vi "KE3706_read_channels_(openvisafirst).vi"(0 "VISA-Ressourcenname":refnum<visa-resource-name>, 7 "Fehler (Eingang, kein Fehler)":errorcluster) -> (12 "Fehler (Ausgang)":errorcluster, 14 "Fehler (Ausgang) 3":errorcluster caption="Fehler (Ausgang)", 18 "Fehler (Ausgang) 6":errorcluster caption="Fehler (Ausgang)", 19 "Display Readings 9":string, 20 "Display Readings":string, 21 "Display Readings 2":string, 22 "Display Readings 3":string, 23 "Display Readings 4":string, 24 "Display Readings 5":string, 25 "Display Readings 6":string, 26 "Display Readings 7":string, 27 "Display Readings 8":string)   [LabVIEW 2020]
panel:
  out "Fehler (Ausgang) 2":errorcluster caption="Fehler (Ausgang)"
  out "Fehler (Ausgang) 9":errorcluster caption="Fehler (Ausgang)"
  out "Fehler (Ausgang) 8":errorcluster caption="Fehler (Ausgang)"
  out "Fehler (Ausgang) 7":errorcluster caption="Fehler (Ausgang)"
  out "Fehler (Ausgang) 5":errorcluster caption="Fehler (Ausgang)"
  out "Fehler (Ausgang) 4":errorcluster caption="Fehler (Ausgang)"
  # "der will eh nie einen Fehler hier ausgeben\nsiehe display da macht er es (manchmal, wenn er will)"
  # "man muss manuel triggern\noder irgendwie mit code\ndas teil ist lustig"
  # "die channel können beide auch ine einem wert ausgegeben werden (mittelwert, wahrscheinlich ka?)\nauf jedenfall muss man darauf achten dass die channel seperat bleiben (?)!\nsollte man das ding überhaupt nutzen\n\nder einzige befehl der keinen error wirft ist gerade drin und selbst mit libs und allem möglicen funktionieren auch keine sample codes aus dem manual\ndas problem mit dem display.gettext() ist dass es sobald das display gelesen wird der automatische trigger ausgeschaltet wird."
  # "^nvm das was jetzt da steht funktioniert auch und funktioniert digital\n\nmuss nur gut voreingestellt werden (jana weiß wie)\n\nEUREKA ES GEHT\n\nGerät function auf mytemp in beiden channels (voreinstellung)"
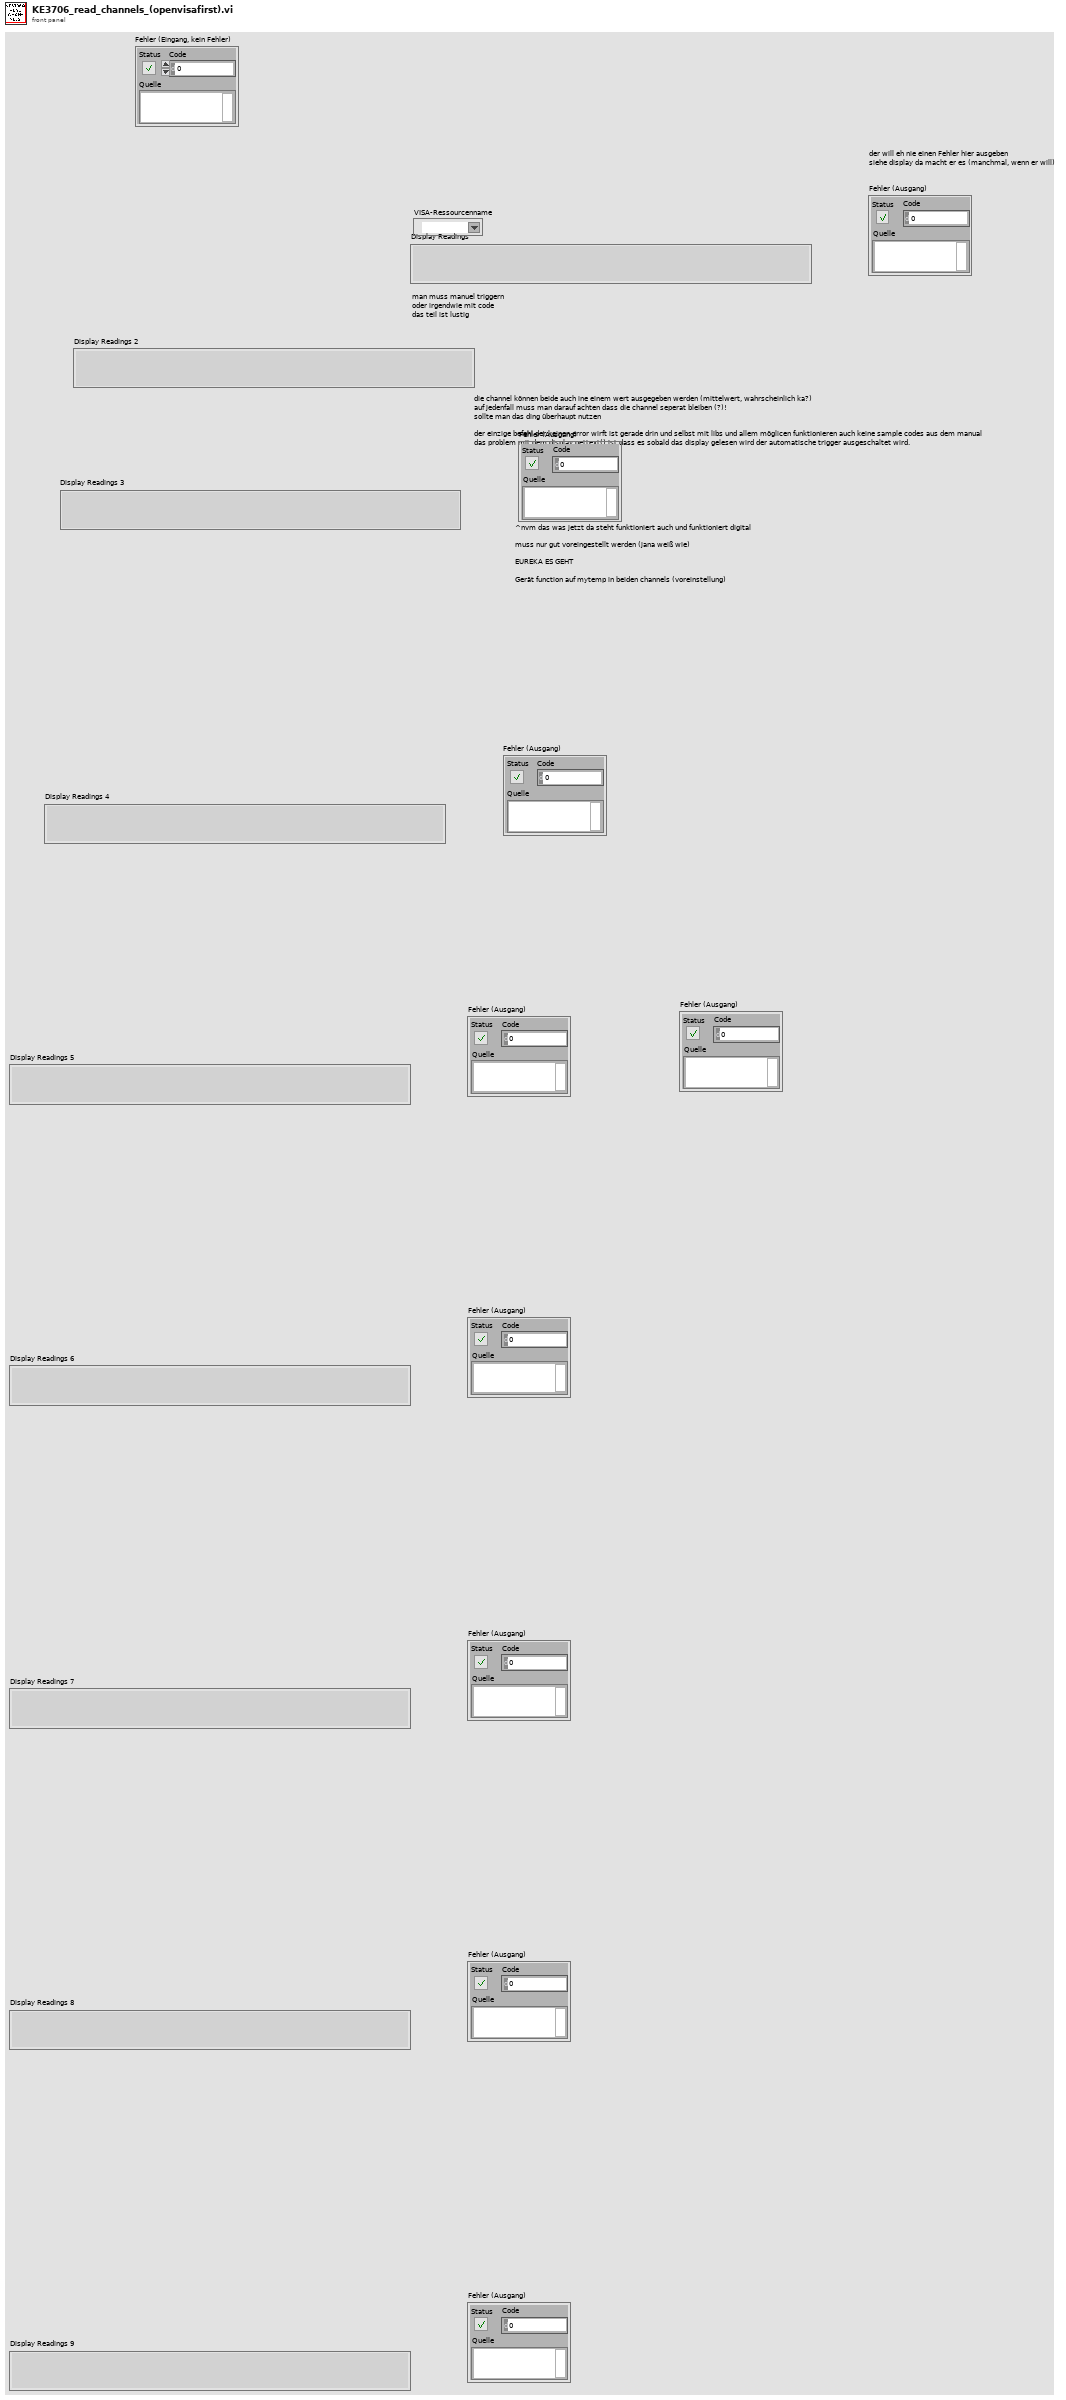
[diagram p1: front panel]
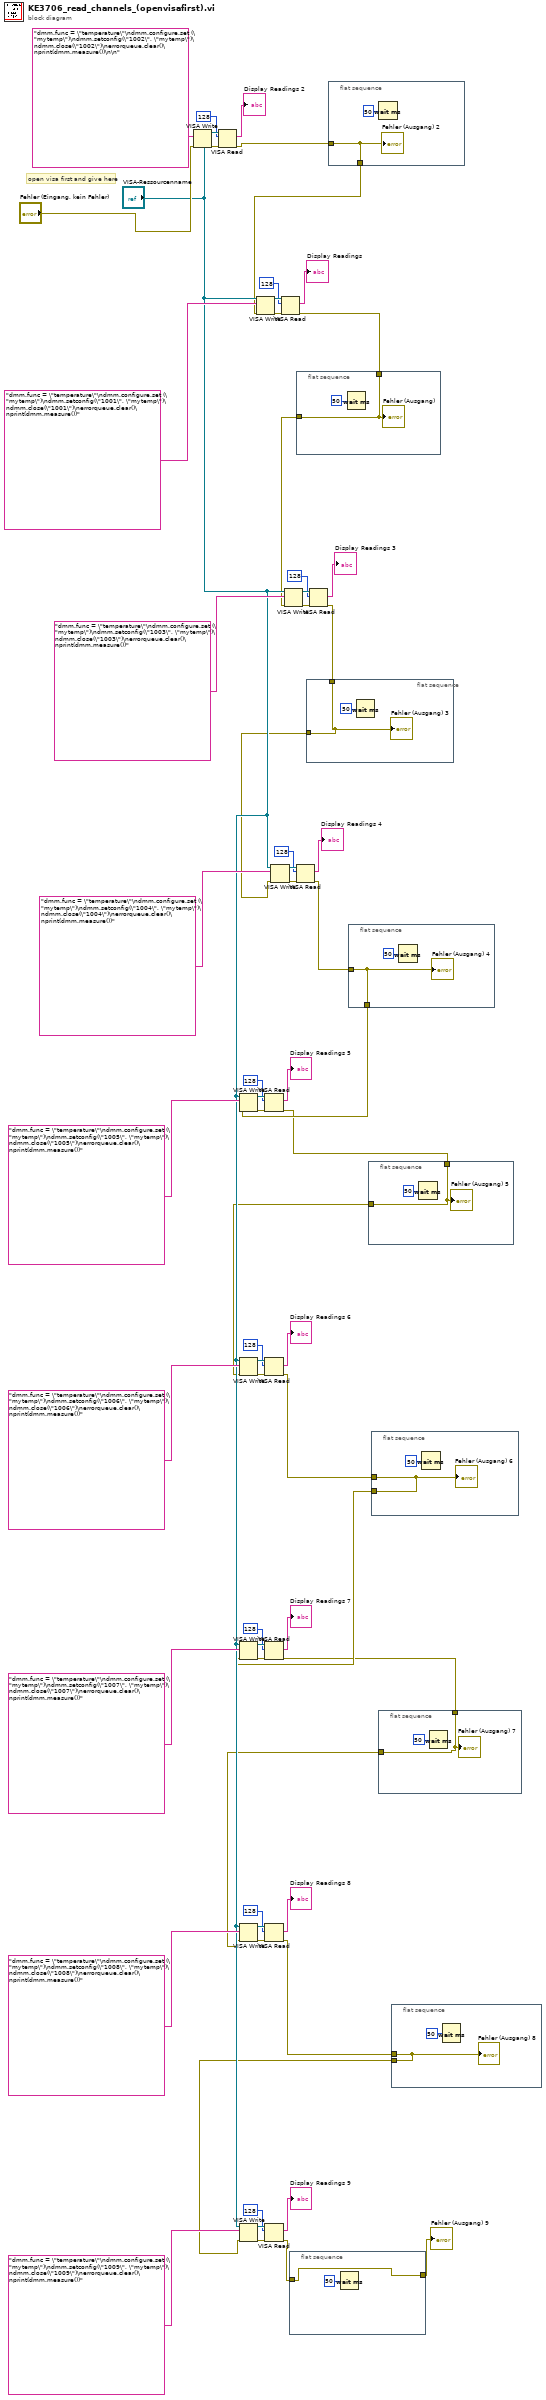
[diagram p0: block diagram]
diagram:
  # "open visa first and give here"
  n1 = VISA Write(VISA resource name="VISA-Ressourcenname", write buffer="dmm.func = \"temperature\"\ndmm.configure.set (\"mytemp\")\ndmm.setconfig(\"1002\", \"mytemp\")\ndmm.close(\"1002\")\nerrorqueue.clear()\nprint(dmm.measure())\n\n" ("Schreibpuffer"), error in (no error)="Fehler (Eingang, kein Fehler)") -> (VISA resource name out=w60:refnum<visa-resource-name>, error out=w59:errorcluster)  [unwired: 1 out]
  n2 = VISA Read(VISA resource name=w60, byte count=u32 128 ("Byte-Anzahl"), error in (no error)=w59) -> (read buffer=→"Display Readings 2":string, error out=w18:errorcluster)  [unwired: 2 out]
  n3 = VISA Write(VISA resource name="VISA-Ressourcenname", write buffer="dmm.func = \"temperature\"\ndmm.configure.set (\"mytemp\")\ndmm.setconfig(\"1005\", \"mytemp\")\ndmm.close(\"1005\")\nerrorqueue.clear()\nprint(dmm.measure())" ("Schreibpuffer"), error in (no error)=w11) -> (VISA resource name out=w44:refnum<visa-resource-name>, error out=w43:errorcluster)  [unwired: 1 out]
  n4 = VISA Write(VISA resource name="VISA-Ressourcenname", write buffer="dmm.func = \"temperature\"\ndmm.configure.set (\"mytemp\")\ndmm.setconfig(\"1006\", \"mytemp\")\ndmm.close(\"1006\")\nerrorqueue.clear()\nprint(dmm.measure())" ("Schreibpuffer"), error in (no error)=w9) -> (VISA resource name out=w39:refnum<visa-resource-name>, error out=w38:errorcluster)  [unwired: 1 out]
  n5 = VISA Write(VISA resource name="VISA-Ressourcenname", write buffer="dmm.func = \"temperature\"\ndmm.configure.set (\"mytemp\")\ndmm.setconfig(\"1007\", \"mytemp\")\ndmm.close(\"1007\")\nerrorqueue.clear()\nprint(dmm.measure())" ("Schreibpuffer"), error in (no error)=w7) -> (VISA resource name out=w34:refnum<visa-resource-name>, error out=w33:errorcluster)  [unwired: 1 out]
  n6 = VISA Write(VISA resource name="VISA-Ressourcenname", write buffer="dmm.func = \"temperature\"\ndmm.configure.set (\"mytemp\")\ndmm.setconfig(\"1008\", \"mytemp\")\ndmm.close(\"1008\")\nerrorqueue.clear()\nprint(dmm.measure())" ("Schreibpuffer"), error in (no error)=w5) -> (VISA resource name out=w29:refnum<visa-resource-name>, error out=w28:errorcluster)  [unwired: 1 out]
  n7 = VISA Write(VISA resource name="VISA-Ressourcenname", write buffer="dmm.func = \"temperature\"\ndmm.configure.set (\"mytemp\")\ndmm.setconfig(\"1009\", \"mytemp\")\ndmm.close(\"1009\")\nerrorqueue.clear()\nprint(dmm.measure())" ("Schreibpuffer"), error in (no error)=w3) -> (VISA resource name out=w24:refnum<visa-resource-name>, error out=w23:errorcluster)  [unwired: 1 out]
  n8 = VISA Write(VISA resource name="VISA-Ressourcenname", write buffer="dmm.func = \"temperature\"\ndmm.configure.set (\"mytemp\")\ndmm.setconfig(\"1001\", \"mytemp\")\ndmm.close(\"1001\")\nerrorqueue.clear()\nprint(dmm.measure())" ("Schreibpuffer"), error in (no error)=w17) -> (VISA resource name out=w65:refnum<visa-resource-name>, error out=w64:errorcluster)  [unwired: 1 out]
  n9 = VISA Read(VISA resource name=w44, byte count=u32 128 ("Byte-Anzahl"), error in (no error)=w43) -> (read buffer=→"Display Readings 5":string, error out=w10:errorcluster)  [unwired: 2 out]
  n10 = VISA Read(VISA resource name=w39, byte count=u32 128 ("Byte-Anzahl"), error in (no error)=w38) -> (read buffer=→"Display Readings 6":string, error out=w8:errorcluster)  [unwired: 2 out]
  n11 = VISA Read(VISA resource name=w34, byte count=u32 128 ("Byte-Anzahl"), error in (no error)=w33) -> (read buffer=→"Display Readings 7":string, error out=w6:errorcluster)  [unwired: 2 out]
  n12 = VISA Read(VISA resource name=w29, byte count=u32 128 ("Byte-Anzahl"), error in (no error)=w28) -> (read buffer=→"Display Readings 8":string, error out=w4:errorcluster)  [unwired: 2 out]
  n13 = VISA Read(VISA resource name=w24, byte count=u32 128 ("Byte-Anzahl"), error in (no error)=w23) -> (read buffer=→"Display Readings 9":string, error out=w2:errorcluster)  [unwired: 2 out]
  n14 = VISA Write(VISA resource name="VISA-Ressourcenname", write buffer="dmm.func = \"temperature\"\ndmm.configure.set (\"mytemp\")\ndmm.setconfig(\"1004\", \"mytemp\")\ndmm.close(\"1004\")\nerrorqueue.clear()\nprint(dmm.measure())" ("Schreibpuffer"), error in (no error)=w13) -> (VISA resource name out=w49:refnum<visa-resource-name>, error out=w48:errorcluster)  [unwired: 1 out]
  n15 = VISA Read(VISA resource name=w65, byte count=u32 128 ("Byte-Anzahl"), error in (no error)=w64) -> (read buffer=→"Display Readings":string, error out=w16:errorcluster)  [unwired: 2 out]
  n16 = VISA Write(VISA resource name="VISA-Ressourcenname", write buffer="dmm.func = \"temperature\"\ndmm.configure.set (\"mytemp\")\ndmm.setconfig(\"1003\", \"mytemp\")\ndmm.close(\"1003\")\nerrorqueue.clear()\nprint(dmm.measure())" ("Schreibpuffer"), error in (no error)=w15) -> (VISA resource name out=w54:refnum<visa-resource-name>, error out=w53:errorcluster)  [unwired: 1 out]
  n17 = flat-sequence {
    tunnel: w2 -> [w66]
    tunnel: [w66] -> w1
    frame #0 {
      n18 = Wait (ms)(milliseconds to wait=u32 50 ("Zu wartende ms")) -> ()  [unwired: 1 out]
    }
  }
  n19 = VISA Read(VISA resource name=w49, byte count=u32 128 ("Byte-Anzahl"), error in (no error)=w48) -> (read buffer=→"Display Readings 4":string, error out=w12:errorcluster)  [unwired: 2 out]
  n20 = flat-sequence {
    tunnel: w16 -> [w68]
    tunnel: [w68] -> w15
    frame #0 {
      n21 = Wait (ms)(milliseconds to wait=u32 50 ("Zu wartende ms")) -> ()  [unwired: 1 out]
      "Fehler (Ausgang)" <- w68
    }
  }
  n22 = flat-sequence {
    tunnel: w14 -> [w70]
    tunnel: [w70] -> w13
    frame #0 {
      n23 = Wait (ms)(milliseconds to wait=u32 50 ("Zu wartende ms")) -> ()  [unwired: 1 out]
      "Fehler (Ausgang) 3" <- w70
    }
  }
  n24 = VISA Read(VISA resource name=w54, byte count=u32 128 ("Byte-Anzahl"), error in (no error)=w53) -> (read buffer=→"Display Readings 3":string, error out=w14:errorcluster)  [unwired: 2 out]
  n25 = flat-sequence {
    tunnel: w18 -> [w72]
    tunnel: [w72] -> w17
    frame #0 {
      n26 = Wait (ms)(milliseconds to wait=u32 50 ("Zu wartende ms")) -> ()  [unwired: 1 out]
      "Fehler (Ausgang) 2" <- w72
    }
  }
  n27 = flat-sequence {
    tunnel: w12 -> [w74]
    tunnel: [w74] -> w11
    frame #0 {
      n28 = Wait (ms)(milliseconds to wait=u32 50 ("Zu wartende ms")) -> ()  [unwired: 1 out]
      "Fehler (Ausgang) 4" <- w74
    }
  }
  n29 = flat-sequence {
    tunnel: w10 -> [w76]
    tunnel: [w76] -> w9
    frame #0 {
      n30 = Wait (ms)(milliseconds to wait=u32 50 ("Zu wartende ms")) -> ()  [unwired: 1 out]
      "Fehler (Ausgang) 5" <- w76
    }
  }
  n31 = flat-sequence {
    tunnel: w8 -> [w78]
    tunnel: [w78] -> w7
    frame #0 {
      n32 = Wait (ms)(milliseconds to wait=u32 50 ("Zu wartende ms")) -> ()  [unwired: 1 out]
      "Fehler (Ausgang) 6" <- w78
    }
  }
  n33 = flat-sequence {
    tunnel: w6 -> [w80]
    tunnel: [w80] -> w5
    frame #0 {
      n34 = Wait (ms)(milliseconds to wait=u32 50 ("Zu wartende ms")) -> ()  [unwired: 1 out]
      "Fehler (Ausgang) 7" <- w80
    }
  }
  n35 = flat-sequence {
    tunnel: w4 -> [w82]
    tunnel: [w82] -> w3
    frame #0 {
      n36 = Wait (ms)(milliseconds to wait=u32 50 ("Zu wartende ms")) -> ()  [unwired: 1 out]
      "Fehler (Ausgang) 8" <- w82
    }
  }
  "Fehler (Ausgang) 9" <- w1
